vi "lab3_1.vi"() -> ()   [LabVIEW 2025]
uses:
  vi/fpga_states.ctl
  <vilib>/rvi/Emulation/niFpgaGetClockAttributes.vi
  <vilib>/rvi/Emulation/niFpgaSctlEmulationGetInTimedLoop.vi
  <vilib>/rvi/Emulation/niFpgaEmulationReportErrorSimple.vi
  <vilib>/rvi/Emulation/niFpgaEmulationIsFPGAContextNoSignature.vi
  <vilib>/rvi/errors/niFpgaSetErrorForExecOnDevCompSimple.vi
  <vilib>/rvi/eio/common/nirviEmuReportErrorAndStop.vi
  <vilib>/rvi/DataTransferAndStorage/Container/Common/niFpgaContainerGetUniqueNameForEmu.vi
  <vilib>/rvi/FIFO/Fifo_Resource/nirvififoEmulationSetSize.vi
  <vilib>/rvi/FIFO/Fifo_Resource/nirviFifoEmulationQueueMgr.vi
  <instcachedir>/0/nirviFifoEmulationQueueMgr_E5CAEC123FF24DC58D834DCA3CDAA9B5.lvgen/nirviFifoEmulationQueueMgr_E5CAEC123FF24DC58D834DCA3CDAA9B5_002.vi
  <vilib>/Utility/error.llb/Clear Errors.vi
  <vilib>/rvi/FIFO/Fifo_Resource/nirvififoEmulationCreateLock.vi
  <vilib>/rvi/Emulation/niFpgaProcessEmulError.vi
  <vilib>/rvi/FIFO/Fifo_Resource/nirvififoEmulationObtainLock.vi
  <vilib>/rvi/FIFO/Fifo_Resource/nirvififoEmulationReleaseLock.vi
  <vilib>/rvi/occurrence/nirviWaitOnOccurrenceBase.vi
  <vilib>/rvi/errors/nirviReportUnexpectedCaseInternalError.vi
  <vilib>/rvi/errors/nirviReportUnexpectedCaseInternalError (U32).vi
  <vilib>/eio/utilities/niEioResolveVilibRelativePath.vi
  <vilib>/rvi/interface/RandomDataEmulation/niFpgaRandomDataHandleErrors.vi
  <vilib>/rvi/Emulation/niFpgaCriticalErrorInLSC.vi
  <vilib>/rvi/eio/common/nirviEmuTemplateMethod_errors.vi
  <vilib>/rvi/FIFO/Fifo_Resource/nirvififoEmulationDetermineInputValidOut.vi
  <vilib>/rvi/DataTransferAndStorage/Container/XNode/niFpgaContainer.xnode
  <vilib>/rvi/FIFO/Fifo_Resource/nirvififoEmulationRead.vi
  <vilib>/rvi/interface/RandomDataEmulation/nirviRandomDataFpgaReadWriteTemplate.vi
  <vilib>/eio/EIONode/EIONode.xnode
  <vilib>/rvi/FIFO/Fifo_Resource/nirvififoEmulationWrite.vi
panel:
  in  "Treshold":i16
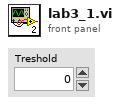
[diagram p1: front panel]
types:
  T1 = typedef "fpga_states.ctl" = enum16{"Wait", "Collect"}
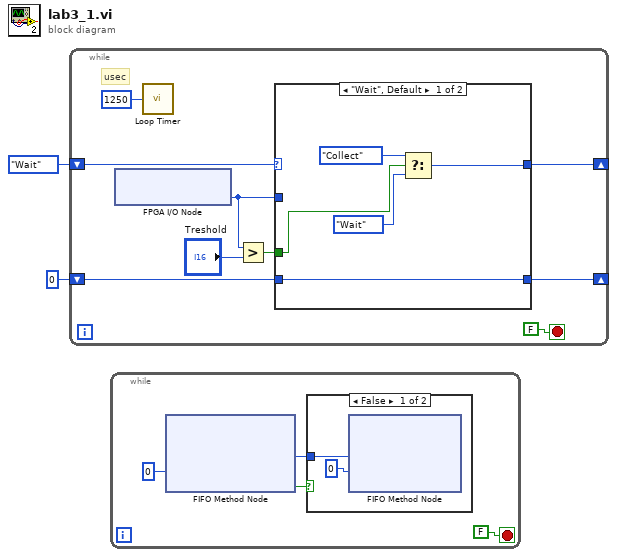
[diagram p0: block diagram]
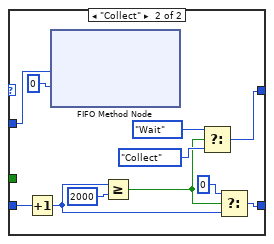
[diagram p3: hidden frame]
diagram:
  n1 = while {
    shift-right: [w6] -> _
    shift-left: fpga_states."Wait" -> [w8]
    shift-right: [w4] -> _
    shift-left: i16 0 -> [w5]
    stop <- FALSE stop-if-true
    # "usec"
    n2 = xnode "FPGA I/O Node"() -> ("AccelerationX"=w3:i16)  [unwired: 1 in, 1 out]
    n3 = call "Loop Timer"("Count(uSec)"=u32 1250) -> ()  [unwired: 1 out]
    n4 = Greater?(x=w3, y="Treshold") -> (0:w7:bool)
    n5 = case shown="\"Wait\", Default" w8 {
      tunnel: w7 -> [w15 _]
      tunnel: [w12 w21] -> w6
      tunnel: w5 -> [w16 w27]
      tunnel: [w16 w17] -> w4
      tunnel: w3 -> [_ w25]
      frame "Wait", Default {
        n6 = Select(t=fpga_states."Collect", s=w15, f=fpga_states."Wait") -> (s? t:f=w12:T1)
      }
      frame "Collect" {
        n7 = Increment(x=w27) -> (x+1=w19:i16)
        n8 = xnode ("FIFO Method Node")("Element"=w25, "Timeout"=0) -> ()  [unwired: 1 in, 2 out]
        n9 = Greater Or Equal?(x=w19, y=i16 2000) -> (x >= y?=w20:bool)
        n10 = Select(t=fpga_states."Wait", s=w20, f=fpga_states."Collect") -> (s? t:f=w21:T1)
        n11 = Select(t=i16 0, s=w20, f=w19) -> (s? t:f=w17:i16)
      }
    }
  }
  n12 = while {
    stop <- FALSE stop-if-true
    n13 = xnode ("FIFO Method Node")("Timeout"=0) -> ("Element"=w30:u64, "Timed Out?"=w31:bool)  [unwired: 1 in, 1 out]
    n14 = case shown="False" w31 {
      tunnel: w30 -> [w32 _]
      frame False {
        n15 = xnode ("FIFO Method Node")("Element"=w32, "Timeout"=0) -> ()  [unwired: 1 in, 2 out]
      }
      frame True {
      }
    }
  }
